vi "Handle Mouse Down.vi"(4 "PlatMods":T1, 5 "VolatusAPI":refnum<class "VolatusAPI.lvclass">, 6 "Mods":cluster{"Double Click":bool, "Menu Key":bool}, 7 "CtlRef":refnum<vi>, 8 "error in (no error)":errorcluster, 9 "Coords":T2, 10 "Button":u16, 11 "DblPopupControl in":refnum<class "DblPopupControl.lvclass">) -> (0 "error out":errorcluster, 3 "DblPopupControl out":refnum<class "DblPopupControl.lvclass">)   [LabVIEW 2020, in "VolatusGUIElements.lvlib" / "DblPopupControl.lvclass"]
uses:
  DblPopupControl.lvclass
  DblPopupControl.lvclass/DblPopupControl.ctl
  Value Prompt Async.vi
  <vilib>/Utility/miscctls.llb/LVPoint32TypeDef.ctl
  Volatus/VolatusAPI/VolatusAPI.lvclass
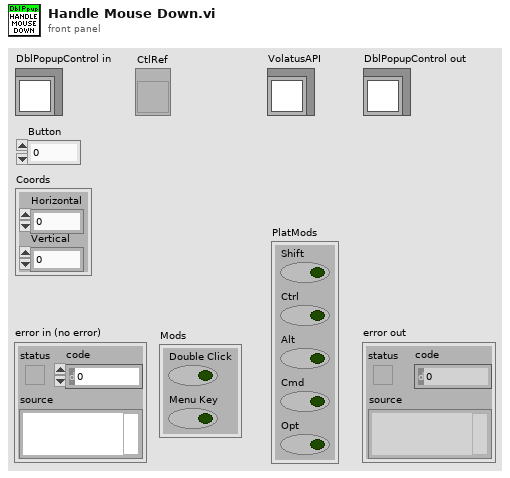
[diagram p1: front panel]
types:
  T1 = cluster{"Shift":bool, "Ctrl":bool, "Alt":bool, "Cmd":bool, "Opt":bool}
  T2 = typedef "LVPoint32TypeDef.ctl" = cluster{"Horizontal":i32, "Vertical":i32}
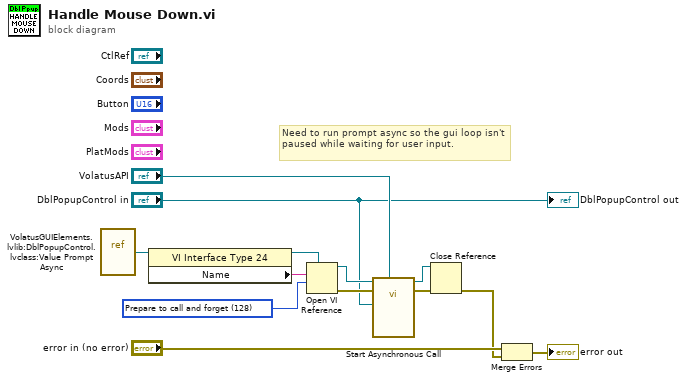
[diagram p0: block diagram]
diagram:
  w7 = 128 items=["Record modifications"=1, "Open templates for editing"=2, "Prompt user to save"=4, "Prepare for reentrant run"=8, "Prompt to find missing subVIs"=16, "Hide loading dialog box"=32, "Enable simultaneous calls"=64, "Prepare to call and forget"=128, "Simultaneous call and forget"=192, "Prepare to call and collect"=256, "Simultaneous call and collect"=320]
  # "Need to run prompt async so the gui loop isn't paused while waiting for user input."
  n1 = vi-ref "VolatusGUIElements.lvlib:DblPopupControl.lvclass:Value Prompt Async.vi"() -> (w5:refnum<vi>)
  n2 = property class="VI Interface Type 24"(reference=w5) -> (reference out=w8:refnum<vi>, "Name"=w6:string)  [unwired: 1 in, 1 out]
  n3 = Open VI Reference(type specifier VI Refnum (for type only)=w8, vi path=w6, options=w7) -> (vi reference=w4:refnum<vi>, error out=w9:errorcluster)  [unwired: 3 in]
  n4 = call-by-ref "Start Asynchronous Call"(reference=w4, error in=w9, "VolatusAPI"="VolatusAPI", "DblPopupControl in"="DblPopupControl in") -> (reference out=w3:refnum<vi>, error out=w2:errorcluster)  [unwired: 10 in]
  n5 = Close Reference(reference=w3, error in (no error)=w2) -> (error out=w11:errorcluster)
  n6 = Merge Errors("error in (no error)", w11) -> (→"error out":errorcluster)
  "DblPopupControl out" <- "DblPopupControl in"
